vi "Game_AI_Move.vi"(0 "Context":T1={"Screen"=enum."Settings", "Settings"=[0, 0, 1, 1], "Board"={"Grid"=array15x15[225 elements], "Move History"=[], "Last Move"={"Row"=-1, "Col"=-1, "Stone"=enum."Empty"}}, "Status"=enum."Idle", "Game ID"=0, "Player Stone"=enum."Black", "Hover"={"Row"=-1, "Col"=-1, "Stone"=enum."Empty"}, "Hover Button"=-1, "Win Line"=[], "Score 1"=0, "Score 2"=0, "Draws"=0, "Status Text"="", "Status Color"=0}, 5 "Move":T2={"Row"=-1, "Col"=-1, "Stone"=enum."Empty"}, 7 "Game ID":u32, 11 "error in":errorcluster) -> (4 "Context out":T1={"Screen"=enum."Settings", "Settings"=[0, 0, 1, 1], "Board"={"Grid"=array15x15[225 elements], "Move History"=[], "Last Move"={"Row"=-1, "Col"=-1, "Stone"=enum."Empty"}}, "Status"=enum."Idle", "Game ID"=0, "Player Stone"=enum."Black", "Hover"={"Row"=-1, "Col"=-1, "Stone"=enum."Empty"}, "Hover Button"=-1, "Win Line"=[], "Score 1"=0, "Score 2"=0, "Draws"=0, "Status Text"="", "Status Color"=0}, 15 "error out":errorcluster)   [LabVIEW 2026]
doc: "AI 착수 결과 반영. Game ID가 현재 판과 같고 AI 차례일 때만 둔다. AI 승리면 Score 2 증가."
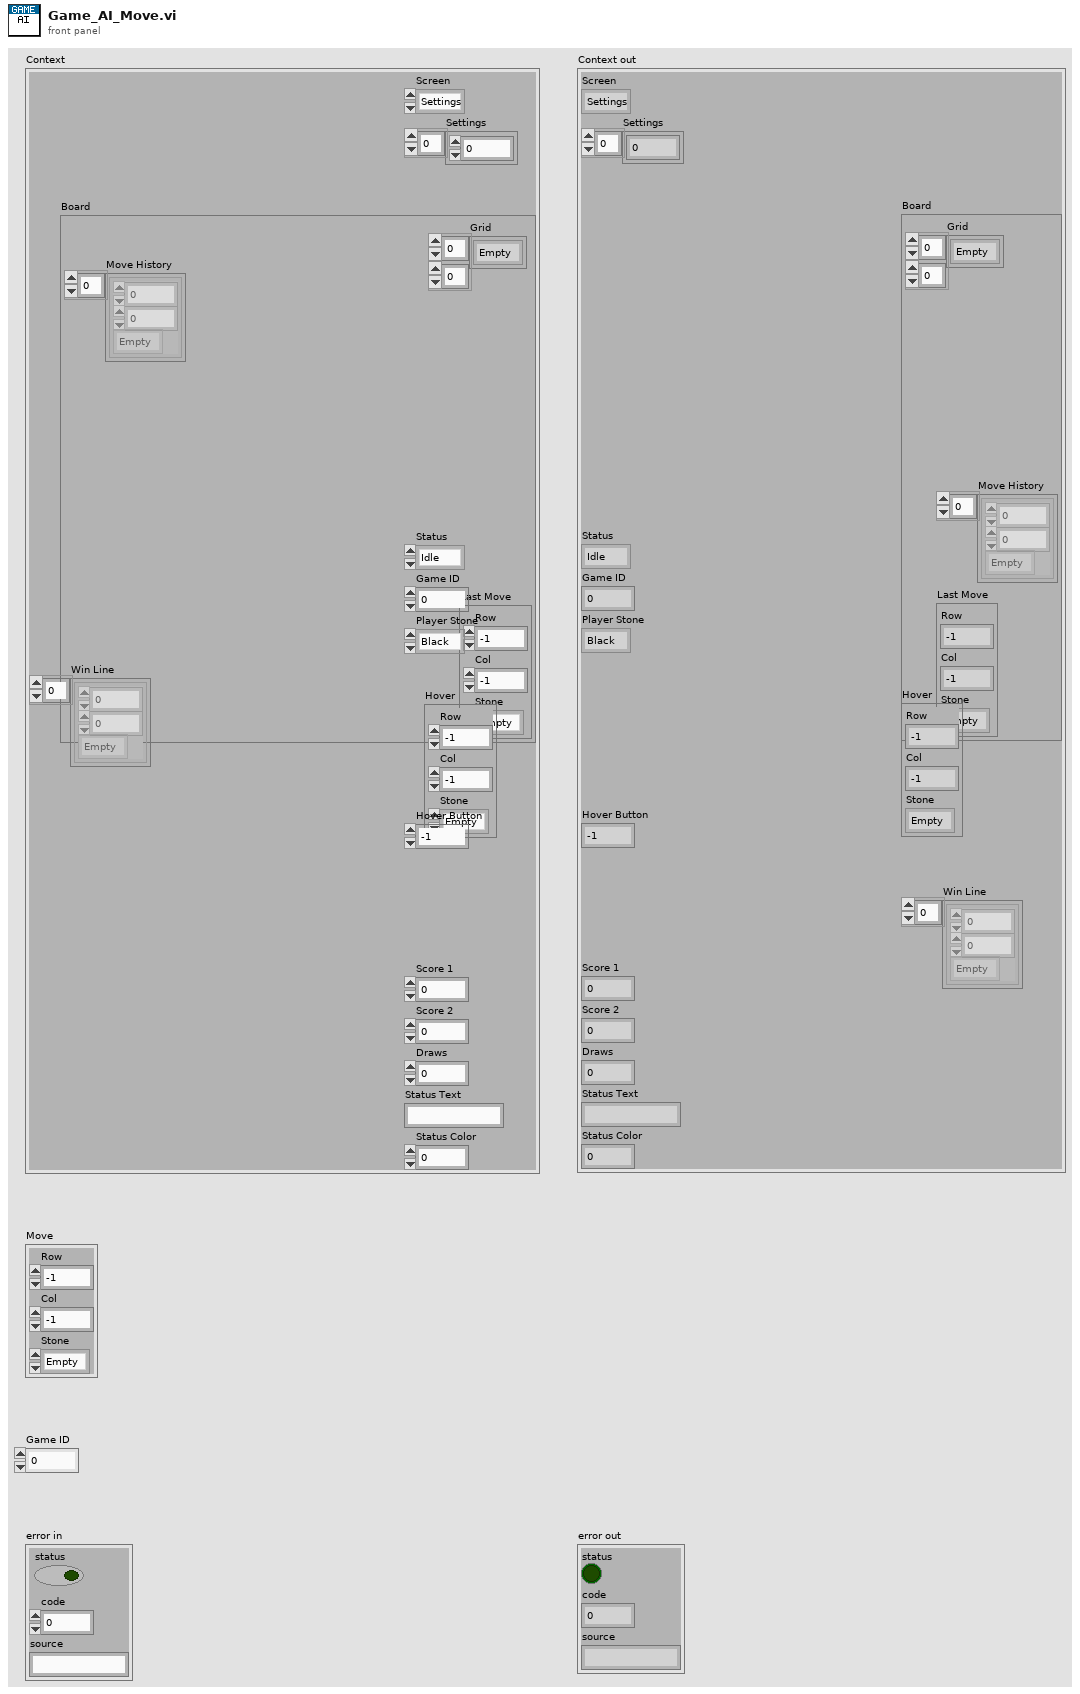
[diagram p1: front panel]
types:
  T1 = cluster{"Screen":enum16{"Settings", "Game"}, "Settings":i32[], "Board":cluster{"Grid":enum8{"Empty", "Black", "White"}[][], "Move History":cluster{"Row":i32, "Col":i32, "Stone":enum8{"Empty", "Black", "White"}}[], "Last Move":cluster{"Row":i32, "Col":i32, "Stone":enum8{"Empty", "Black", "White"}}}, "Status":enum16{"Idle", "Player Turn", "AI Thinking", "Game Over"}, "Game ID":u32, "Player Stone":enum8{"Empty", "Black", "White"}, "Hover":cluster{"Row":i32, "Col":i32, "Stone":enum8{"Empty", "Black", "White"}}, "Hover Button":i32, "Win Line":cluster{"Row":i32, "Col":i32, "Stone":enum8{"Empty", "Black", "White"}}[], "Score 1":i32, "Score 2":i32, "Draws":i32, "Status Text":string, "Status Color":u32}
  T2 = cluster{"Row":i32, "Col":i32, "Stone":enum8{"Empty", "Black", "White"}}
  T3 = enum16{"Idle", "Player Turn", "AI Thinking", "Game Over"}
  T4 = cluster{"Grid":enum8{"Empty", "Black", "White"}[][], "Move History":cluster{"Row":i32, "Col":i32, "Stone":enum8{"Empty", "Black", "White"}}[], "Last Move":cluster{"Row":i32, "Col":i32, "Stone":enum8{"Empty", "Black", "White"}}}
  T5 = cluster{"Row":i32, "Col":i32, "Stone":enum8{"Empty", "Black", "White"}}[]
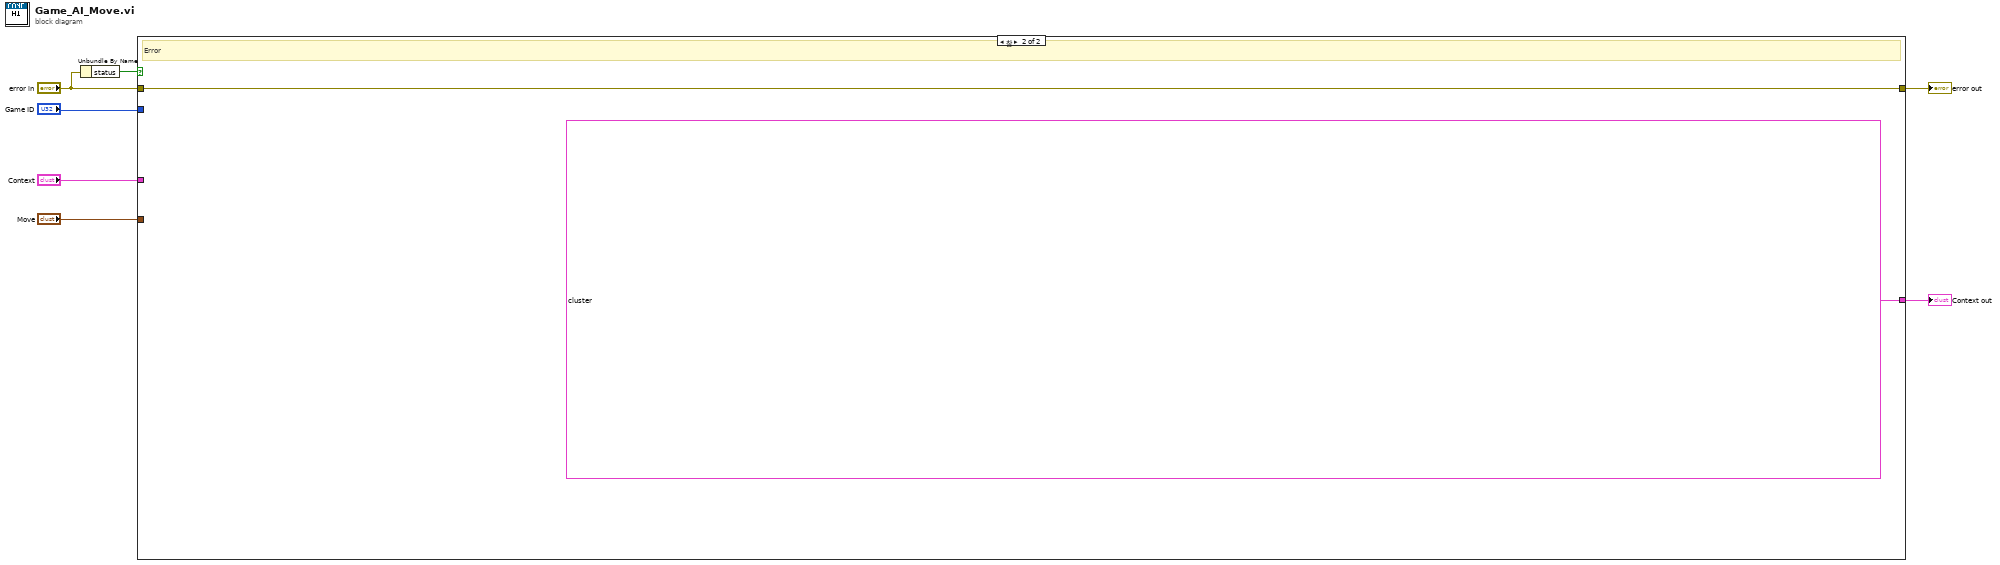
[diagram p0: block diagram]
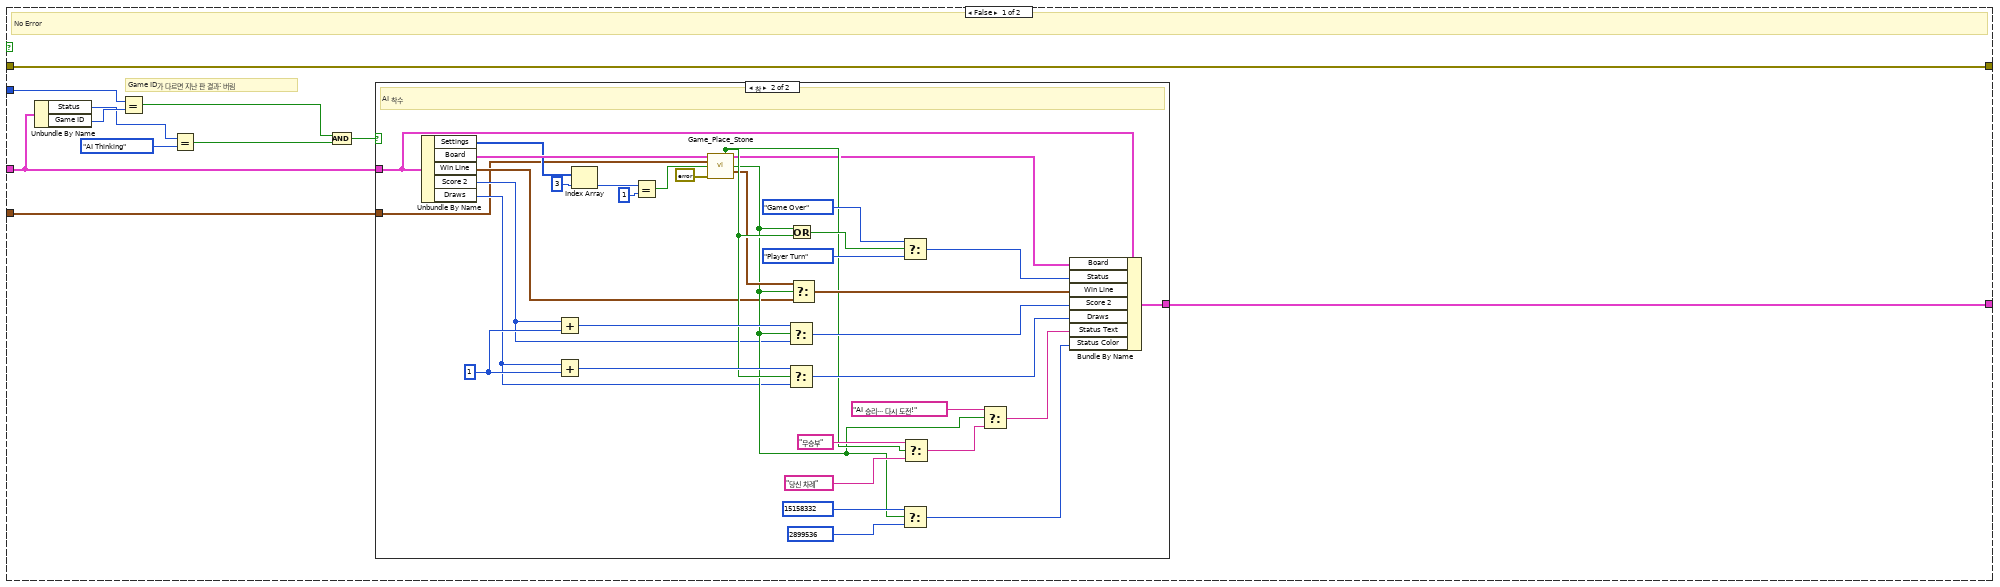
[diagram p2: hidden frame]
diagram:
  n1 = Unbundle By Name("error in") -> ("status"=w5:bool)
  n2 = case shown="참" w5 {
    tunnel: "Context" -> [w8 _]
    tunnel: "Move" -> [w9 _]
    tunnel: "Game ID" -> [w10 _]
    tunnel: "error in" -> [w11 w55]
    tunnel: [w11 w55] -> w7
    tunnel: [w18 T1 {"Screen"=enum."Settings", "Settings"=[0, 0, 1, 1], "Board"={"Grid"=array15x15[225 elements], "Move History"=[], "Last Move"={"Row"=-1, "Col"=-1, "Stone"=enum."Empty"}}, "Status"=enum."Idle", "Game ID"=0, "Player Stone"=enum."Black", "Hover"={"Row"=-1, "Col"=-1, "Stone"=enum."Empty"}, "Hover Button"=-1, "Win Line"=[], "Score 1"=0, "Score 2"=0, "Draws"=0, "Status Text"="", "Status Color"=0}] -> w6
    frame False {
      # "Game ID가 다르면 지난 판 결과: 버림"
      # "No Error"
      n3 = Unbundle By Name(w8) -> ("Status"=w12:T3, "Game ID"=w13:u32)
      n4 = Equal?(x=w10, y=w13) -> (x = y?=w14:bool)
      n5 = Equal?(x=w12, y=T3."AI Thinking") -> (x = y?=w16:bool)
      n6 = And(x=w14, y=w16) -> (x .and. y?=w17:bool)
      n7 = case shown="참" w17 {
        tunnel: w8 -> [w19 w20]
        tunnel: w9 -> [_ w21]
        tunnel: [w19 w54] -> w18
        frame False {
          # "버림"
        }
        frame True {
          w37 = 1
          # "AI 착수"
          n8 = Unbundle By Name(w20) -> ("Settings"=w22:i32[], "Board"=w23:T4, "Win Line"=w24:T5, "Score 2"=w25:i32, "Draws"=w26:i32)
          n9 = Add(x=w25, y=w37) -> (x+y=w50:i32)
          n10 = Add(x=w26, y=w37) -> (x+y=w52:i32)
          n11 = Index Array(array=w22, index=3) -> (element=w28:i32)
          n12 = Equal?(x=w28, y=1) -> (x = y?=w30:bool)
          n13 = call "Game_Place_Stone.vi"("Board State"=w23, "Move"=w21, "Renju"=w30, "error in"=errorcluster {"status"=FALSE, "code"=0, "source"=""}) -> ("Draw?"=w35:bool, "Board State out"=w32:T4, "Win?"=w33:bool, "Win Line"=w34:T5)  [unwired: 5 in, 3 out]
          n14 = Select(t=w50, s=w33, f=w25) -> (s? t:f=w51:i32)
          n15 = Select(t=w52, s=w35, f=w26) -> (s? t:f=w53:i32)
          n16 = Or(x=w33, y=w35) -> (x .or. y?=w36:bool)
          n17 = Select(t=w34, s=w33, f=w24) -> (s? t:f=w49:T5)
          n18 = Select(t=T3."Game Over", s=w36, f=T3."Player Turn") -> (s? t:f=w48:T3)
          n19 = Select(t=u32 15158332, s=w33, f=u32 2899536) -> (s? t:f=w45:u32)
          n20 = Select(t="무승부", s=w35, f="당신 차례") -> (s? t:f=w41:string)
          n21 = Select(t="AI 승리... 다시 도전!", s=w33, f=w41) -> (s? t:f=w42:string)
          n22 = Bundle By Name(cluster=w20, "Board"=w32, "Status"=w48, "Win Line"=w49, "Score 2"=w51, "Draws"=w53, "Status Text"=w42, "Status Color"=w45) -> (w54:T1)
        }
      }
    }
    frame True {
      # "Error"
    }
  }
  "Context out" <- w6
  "error out" <- w7
